vi "Tree -- Cron Library.vi"() -> ()   [LabVIEW 2013]
uses:
  JobReport/JobReport.lvclass
  JobReport/JobReport.lvclass/JobReport.ctl
  Job/Job Report -- cluster.ctl
  Job/Job.lvclass
  Job/Job Update -- cluster.ctl
  Job/Job Started -- cluster.ctl
  Job/Job.lvclass/Job.ctl
  Cron.Jenkins/Cron.Jenkins.lvclass/Cron.Jenkins.ctl
  Cron.Quartz/Cron.Quartz.lvclass
  Cron.Unix/Cron.Unix.lvclass
  Cron.Jenkins/Cron.Jenkins.lvclass
  Cron/Cron.lvclass/Cron.ctl
  Job/Read Abort Notifier.vi
  Cron.Jenkins/Write Job Name.vi
  <vilib>/Utility/error.llb/Error Cluster From Error Code.vi
  Cron/Cron.lvclass
  openCron.lvlib
  Job.StaticVIRef/Job.StaticVIRef.lvclass
panel:
  out "Next Occurence 3":timestamp
  out "syntax valid? (Jenkins)":bool
  out "Next Occurence 2":timestamp
  out "syntax valid? (Unix)":bool
  out "syntax valid? (Quartz)":bool
  out "Next Occurence":timestamp
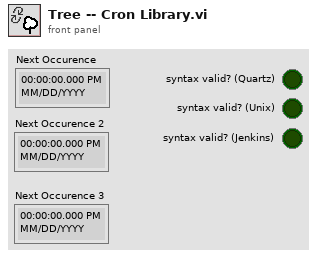
[diagram p1: front panel]
types:
  T1 = typedef "openCronJob.lvlib/Job.lvclass/Job Update -- cluster.ctl" = cluster{"Name":string, "GUID":string, "Time Stamp":timestamp, "Status Message":string, "% Complete":dbl}
  T2 = typedef "openCronJob.lvlib/Job.lvclass/Job Started -- cluster.ctl" = cluster{"Name":string, "GUID":string, "Time Stamp":timestamp}
  T3 = typedef "openCronJob.lvlib/JobReport.lvclass/Job Report -- cluster.ctl" = cluster{"Name":string, "GUID":string, "Start Time":timestamp, "Duration (s)":dbl, "exception code":i32, "stdin":string, "stdout":string}
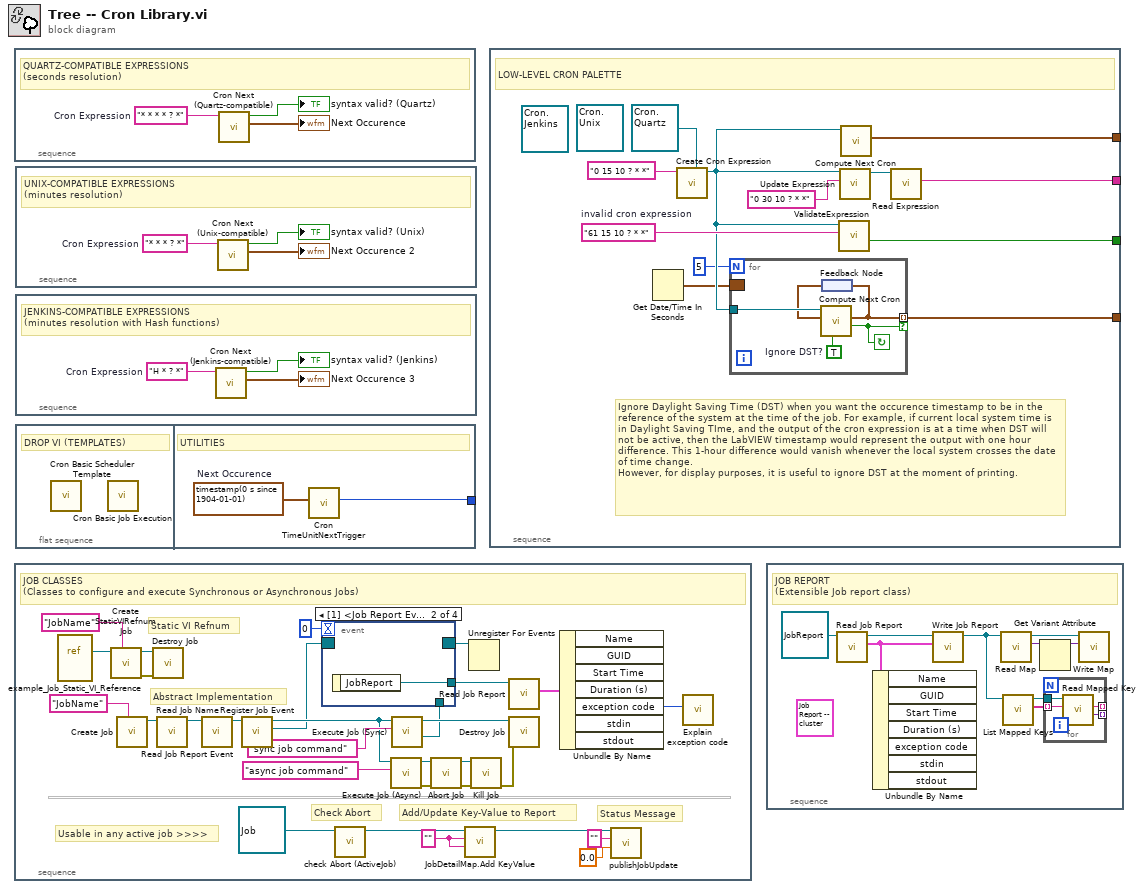
[diagram p0: block diagram]
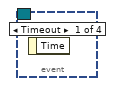
[diagram p2: hidden frame]
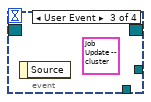
[diagram p3: hidden frame]
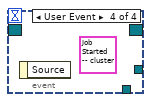
[diagram p4: hidden frame]
diagram:
  n1 = stacked-sequence {
    frame #0 {
      w3 = "* * * * ? *"  # Cron Expression
      # "QUARTZ-COMPATIBLE EXPRESSIONS\n(seconds resolution)"
      n2 = call "Cron Next (Quartz-compatible).vi"("Cron Expression"=w3) -> ("Next Occurence"=→"Next Occurence":timestamp, "syntax valid?"=→"syntax valid? (Quartz)":bool)  [unwired: 8 in, 1 out]
    }
  }
  n3 = stacked-sequence {
    frame #0 {
      w7 = "" ("Key")
      # "Status Message"
      # "Add/Update Key-Value to Report"
      # "Check Abort"
      # "Usable in any active job >>>>"
      # "Abstract Implementation"
      # "Static VI Refnum"
      # "JOB CLASSES\n(Classes to configure and execute Synchronous or Asynchronous Jobs)"
      n4 = vi-ref "example_Job_Static_VI_Reference.vi"() -> (w17:refnum<vi>)
      n5 = call "Create StaticVIRefnum Job.vi"("Job Name"="JobName", "Static VI Refnum"=w17) -> ("error out"=w18:errorcluster, "Job.StaticVIRef out"=w19:refnum<class "Job.StaticVIRef.lvclass">)  [unwired: 8 in]
      n6 = call "Create Job.vi"("Job Name"="JobName") -> ("Job"=w32:refnum<class "Job.lvclass">)  [unwired: 9 in, 1 out]
      n7 = call "Destroy Job.vi"("error in (no error)"=w18, "Job in"=w19) -> ()  [unwired: 8 in, 2 out]
      n8 = call "Read Job Name.vi"("Job in"=w32) -> ("Job out"=w28:refnum<class "Job.lvclass">)  [unwired: 8 in, 2 out]
      n9 = call "Read Job Report Event.vi"("Job in"=w28) -> ("Job out"=w27:refnum<class "Job.lvclass">)  [unwired: 6 in, 4 out]
      n10 = call "Register Job Event.vi"("Job in"=w27) -> ("Job Event Registration"=w24:refnum<event-registration>, "Job out"=w29:refnum<class "Job.lvclass">)  [unwired: 9 in]
      n11 = call "check Abort (ActiveJob).vi"("Job in"=refnum<class "Job.lvclass"> refnum) -> ("Job out"=w8:refnum<class "Job.lvclass">)  [unwired: 7 in, 3 out]
      n12 = call "Execute Job (Async).vi"("stdin"="async job command" ("Job Name"), "Job in"=w29) -> ("error out"=w12:errorcluster, "Job out"=w26:refnum<class "Job.lvclass">)  [unwired: 7 in, 1 out]
      n13 = call "Execute Job (Sync).vi"("stdin"="sync job command" ("Job Name"), "Job in"=w29) -> ("JobReport"=w15:refnum<class "JobReport.lvclass">, "Job out"=w21:refnum<class "Job.lvclass">)  [unwired: 6 in, 2 out]
      n14 = event shown="[1] <Job Report Event>: User Event" {
        selector: w24 -> [_ _ _ _]
        dyn-events: [_ _ _ _] -> w23
        timeout: 0 -> [_ _ _ _]
        tunnel: [_ w34 _ _] -> w10
        tunnel: w15 -> [_ _ _ _]
        event Timeout {
          n15 = event-data() -> ()  [unwired: 1 in, 1 out]
        }
        event User Event {
          n16 = event-data() -> ("JobReport"=w34:refnum<class "JobReport.lvclass">)  [unwired: 1 in]
        }
        event User Event {
          (unwired) T1 {"Name"="", "GUID"="", "Time Stamp"=timestamp(0 s since 1904-01-01), "Status Message"="", "% Complete"=nan} ("Job Update")
          n17 = event-data() -> ()  [unwired: 1 in, 1 out]
        }
        event User Event {
          (unwired) T2 {"Name"="", "GUID"="", "Time Stamp"=timestamp(0 s since 1904-01-01)} ("Job Started")
          n18 = event-data() -> ()  [unwired: 1 in, 1 out]
        }
      }
      n19 = call "Abort Job.vi"("error in (no error)"=w12, "Job in"=w26) -> ("error out"=w13:errorcluster, "Job out"=w25:refnum<class "Job.lvclass">)  [unwired: 5 in, 3 out]
      n20 = call "JobDetailMap.Add KeyValue.vi"("Value"=w7, "Key"=w7, "Job in"=w8) -> ("Job out"=w6:refnum<class "Job.lvclass">)  [unwired: 7 in, 1 out]
      n21 = Unregister For Events(event registration refnum=w23) -> ()  [unwired: 1 in, 1 out]
      n22 = call "Kill Job.vi"("error in (no error)"=w13, "Job in"=w25) -> ("error out"=w14:errorcluster)  [unwired: 8 in, 1 out]
      n23 = call "Read Job Report.vi"("JobReport in"=w10) -> ("Job Report"=w11:T3)  [unwired: 8 in, 2 out]
      n24 = call "Destroy Job.vi"("error in (no error)"=w14, "Job in"=w21) -> ()  [unwired: 8 in, 2 out]
      n25 = Unbundle By Name(w11) -> ("exception code"=w20:i32)  [unwired: 6 out]
      n26 = call "publishJobUpdate.vi"("% Complete (NaN if unknown)"=0.0, "Status Message"="", "Job in"=w6) -> ()  [unwired: 7 in, 2 out]
      n27 = call "Explain exception code.vi"("exception"=w20) -> ()  [unwired: 8 in, 3 out]
    }
  }
  n28 = stacked-sequence {
    frame #0 {
      w37 = "* * * ? *"  # Cron Expression
      # "UNIX-COMPATIBLE EXPRESSIONS\n(minutes resolution)"
      n29 = call "Cron Next (Unix-compatible).vi"("Cron Expression"=w37) -> ("Next Occurence"=→"Next Occurence 2":timestamp, "syntax valid?"=→"syntax valid? (Unix)":bool)  [unwired: 8 in, 1 out]
    }
  }
  n30 = stacked-sequence {
    frame #0 {
      w40 = "H * ? *"  # Cron Expression
      # "JENKINS-COMPATIBLE EXPRESSIONS\n(minutes resolution with Hash functions)"
      n31 = call "Cron Next (Jenkins-compatible).vi"("Cron Expression"=w40) -> ("Next Occurence"=→"Next Occurence 3":timestamp, "syntax valid?"=→"syntax valid? (Jenkins)":bool)  [unwired: 8 in, 1 out]
    }
  }
  n32 = flat-sequence {
    tunnel: [w41] -> _
    frame #0 {
      # "DROP VI (TEMPLATES)"
      n33 = call "Cron Basic Scheduler Template.vi"() -> ()  [unwired: 12 in]
      n34 = call "Cron Basic Job Execution.vi"() -> ()  [unwired: 12 in]
    }
    frame #1 {
      w42 = timestamp(0 s since 1904-01-01)  # Next Occurence
      # "UTILITIES"
      n35 = call "Cron TimeUnitNextTrigger.vi"("Next Occurence"=w42) -> ("next event (ms)"=w41:i32)  [unwired: 10 in]
    }
  }
  n36 = stacked-sequence {
    tunnel: [w46] -> _
    tunnel: [w45] -> _
    tunnel: [w44] -> _
    tunnel: [w43] -> _
    frame #0 {
      (unwired) refnum<class "Cron.Jenkins.lvclass"> refnum ("Cron.Jenkins")
      w52 = "61 15 10 ? * *"  # invalid cron expression
      (unwired) refnum<class "Cron.Unix.lvclass"> refnum ("openCron.lvlib:Cron.Unix.lvclass")
      # "Ignore Daylight Saving Time (DST) when you want the occurence timestamp to be in the reference of the system at the time of the job. For example, if current local system time is in Daylight Saving TIme, and the output of the cron expression is at a time when DST will not be active, then the LabVIEW timestamp would represent the output with one hour difference. This 1-hour difference would vanish whenever the local system crosses the date of time change.\nHowever, for display purposes, it is useful to ignore DST at the moment of printing."
      # "LOW-LEVEL CRON PALETTE"
      n37 = Get Date/Time In Seconds() -> (seconds since 1Jan1904=w48:timestamp)
      n38 = call "Create Cron Expression.vi"("Cron in"=refnum<class "Cron.Quartz.lvclass"> refnum ("openCron.lvlib:Cron.Quartz.lvclass"), "Cron Expression"="0 15 10 ? * *") -> ("Cron out"=w49:refnum<class "Cron.Quartz.lvclass">)  [unwired: 7 in, 2 out]
      n39 = for {
        N: 5 -> [_]
        tunnel: [w57] -> w44 mode=indexing if=w59
        tunnel: w49 -> [w58]
        border: w48 -> [_]
        stop <- w59 continue-if-true
        w55 = TRUE  # Ignore DST?
        n40 = feedback #1() -> (w56:timestamp)
        n41 = call "Compute Next Cron.vi"("Ignore DST?"=w55, "Time Stamp (Now)"=w56, "Cron in"=w58) -> ("Occurence found"=w59:bool, "Next Occurence"=w57:timestamp)  [unwired: 5 in, 2 out]
        n42 = feedback-in #1(w57) -> ()
      }
      n43 = call "ValidateExpression.vi"("Expression"=w52, "Cron in"=w49) -> ("valid?"=w43:bool)  [unwired: 6 in, 3 out]
      n44 = call "Update Expression.vi"("Expression"="0 30 10 ? * *", "Cron in"=w49) -> ("Cron out"=w50:refnum<class "Cron.Quartz.lvclass">)  [unwired: 7 in, 2 out]
      n45 = call "Compute Next Cron.vi"("Cron in"=w49) -> ("Next Occurence"=w45:timestamp)  [unwired: 7 in, 3 out]
      n46 = call "Read Expression.vi"("Cron in"=w50) -> ("Expression"=w46:string)  [unwired: 8 in, 2 out]
    }
  }
  n47 = stacked-sequence {
    frame #0 {
      (unwired) T3 {"Name"="", "GUID"="", "Start Time"=timestamp(0 s since 1904-01-01), "Duration (s)"=0.0, "exception code"=0, "stdin"="", "stdout"=""} ("Job Report")
      # "JOB REPORT\n(Extensible Job report class)"
      n48 = call "Read Job Report.vi"("JobReport in"=refnum<class "JobReport.lvclass"> refnum ("openCronJob.lvlib:JobReport.lvclass")) -> ("Job Report"=w66:T3, "JobReport out"=w67:refnum<class "JobReport.lvclass">)  [unwired: 8 in, 1 out]
      n49 = Unbundle By Name(w66) -> ()  [unwired: 7 out]
      n50 = call "Write Job Report.vi"("Job Report"=w66, "JobReport in"=w67) -> ("JobReport out"=w62:refnum<class "JobReport.lvclass">)  [unwired: 8 in, 1 out]
      n51 = call "Read Map.vi"("JobReport in"=w62) -> ("Map"=w64:variant, "JobReport out"=w65:refnum<class "JobReport.lvclass">)  [unwired: 8 in, 1 out]
      n52 = call "List Mapped Keys.vi"("JobReport in"=w62) -> ("Mapped Keys"=w60:string[], "JobReport out"=w61:refnum<class "JobReport.lvclass">)  [unwired: 8 in, 1 out]
      n53 = Get Variant Attribute(Variant=w64) -> (duplicate Variant=w63:variant)  [unwired: 3 in, 3 out]
      n54 = for {
        tunnel: w61 -> [w72]
        tunnel: w60 -> [w71] mode=indexing
        tunnel: [w70] -> _ mode=indexing
        tunnel: [w69] -> _ mode=indexing
        n55 = call "Read Mapped Key.vi"("Key"=w71, "JobReport in"=w72) -> ("Value"=w69:variant, "Key dup"=w70:string)  [unwired: 5 in, 3 out]
      }
      n56 = call "Write Map.vi"("Map"=w63, "JobReport in"=w65) -> ()  [unwired: 8 in, 2 out]
    }
  }
